vi "Create String Input Channels.vi"(8 "error in (no error)":errorcluster, 11 "Modbus in":refnum<class "Modbus.lvclass">) -> (0 "error out":errorcluster, 1 "Channels to remove":string[](array[string]), 3 "Modbus out":refnum<class "Modbus.lvclass">)   [LabVIEW 2026, in "Modbus.lvlib" / "Modbus.lvclass"]
uses:
  Modbus.lvclass
  C:/Program Files/National Instruments/LabVIEW 2026/vi.lib/FlexLogger/SDK/PluginSDK.lvlibp/PEFClasses/SDK/Plugin/Plugin.lvclass
  Modbus.lvclass/Modbus.ctl
  Globals/Modbus Strings.vi
  <vilib>/FlexLogger/SDK/PluginSDK.lvlibp/PEFClasses/SDK/Plugin/ParameterAccess/Read I32.vi
  <vilib>/FlexLogger/SDK/PluginSDK.lvlibp/PEFClasses/SDK/Channel/Channel.lvclass
  C:/Program Files/National Instruments/LabVIEW 2026/vi.lib/FlexLogger/SDK/PluginSDK.lvlibp/PEFClasses/SDK/Processing Element/Processing Element.lvclass
  D:/Work/FlexLogger/Features/Modbus Plugin/Modbus - Working Copy/Modbus/Modbus.lvclass
  <vilib>/FlexLogger/SDK/PluginSDK.lvlibp/PEFClasses/SDK/Plugin/Plugin.lvclass
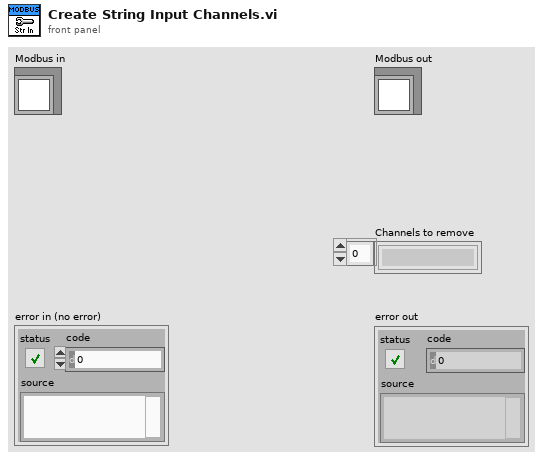
[diagram p1: front panel]
types:
  T1 = typedef "Modbus.lvlib/Modbus.lvclass/String Data.ctl" = cluster{"Channel UID":string, "Valid?":bool, "Table":T2, "Address":i32, "Quantity":u16}
  T2 = typedef "Modbus.lvlib/Modbus.lvclass/Modbus Table.ctl" = enum16{"Discrete Inputs", "Coils", "Input Registers", "Holding Registers"}
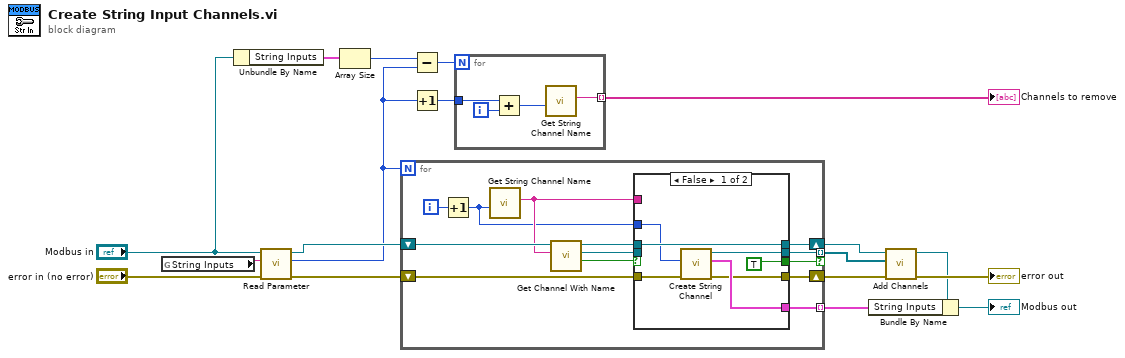
[diagram p0: block diagram]
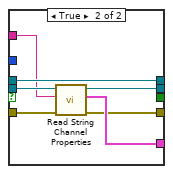
[diagram p2: hidden frame]
diagram:
  n1 = global read "Modbus Strings.vi" "String Inputs"() -> (w10:string)
  n2 = Unbundle By Name("Modbus in") -> ("String Inputs"=w11:T1[])
  n3 = call-poly <vilib>:"Read Parameter.vi"("error in (no error)"="error in (no error)", "Name"=w10, "Plugin in"="Modbus in") -> ("error out"=w13:errorcluster, "Value"=w12:i32, "Plugin out"=w14:refnum<class "Modbus.lvclass">)  [unwired: 5 in, 1 out]
  n4 = Array Size(array=w11) -> (size(s)=w3:i32)
  n5 = for {
    N: w12 -> [_]
    tunnel: [w29] -> w5 mode=indexing if=w28
    shift-right: [w27] -> w6
    shift-left: w13 -> [w26]
    shift-right: [w21] -> w4
    shift-left: w14 -> [w31]
    tunnel: [w25] -> w15 mode=indexing
    i -> [w24]
    n6 = Increment(x=w24) -> (x+1=w19:i32)
    n7 = call "Get String Channel Name.vi"("Channel Numer"=w19) -> ("Bool Channel ID"=w30:string)  [unwired: 9 in, 1 out]
    n8 = call <vilib>:"Get Channel With Name.vi"("Name"=w30, "Plugin in"=w31) -> ("Found?"=w20:bool, "Channel"=w23:refnum<class "Channel.lvclass">, "Plugin out"=w22:refnum<class "Modbus.lvclass">)  [unwired: 7 in]
    n9 = case shown="False" w20 {
      tunnel: w30 -> [_ w39]
      tunnel: [w34 w41] -> w29
      tunnel: [TRUE _] -> w28
      tunnel: [w33 w40] -> w27
      tunnel: w26 -> [w37 w44]
      tunnel: [w36 w43] -> w25
      tunnel: w23 -> [_ w45]
      tunnel: w22 -> [w35 w42]
      tunnel: [w35 w42] -> w21
      tunnel: w19 -> [w32 _]
      frame False {
        n10 = call "Create String Channel.vi"("error in (no error)"=w37, "Channel Number"=w32) -> ("error out"=w33:errorcluster, "Boolean Channel"=w36:T1, "Channel out"=w34:refnum<class "Channel.lvclass">)  [unwired: 7 in]
      }
      frame True {
        n11 = call "Read String Channel Properties.vi"("error in (no error)"=w44, "String Channel ID"=w39, "Channel in"=w45) -> ("error out"=w40:errorcluster, "String Channel"=w43:T1, "Channel out"=w41:refnum<class "Channel.lvclass">)  [unwired: 6 in]
      }
    }
  }
  n12 = Subtract(x=w3, y=w12) -> (x-y=w2:i32)
  n13 = Increment(x=w12) -> (x+1=w1:i32)
  n14 = for {
    N: w2 -> [_]
    tunnel: [w47] -> w17 mode=indexing
    tunnel: w1 -> [w48]
    i -> [w49]
    n15 = Add(x=w48, y=w49) -> (x+y=w46:i32)
    n16 = call "Get String Channel Name.vi"("Channel Numer"=w46) -> ("Bool Channel ID"=w47:string)  [unwired: 9 in, 1 out]
  }
  "Channels to remove" <- w17
  n17 = call <vilib>:"Add Channels.vi"("error in (no error)"=w6, "Channels"=w5, "Plugin in"=w4) -> ("error out"=→"error out":errorcluster, "Plugin out"=w8:refnum<class "Modbus.lvclass">)  [unwired: 7 in]
  n18 = Bundle By Name(cluster=w8, "String Inputs"=w15) -> (→"Modbus out":refnum<class "Modbus.lvclass">)
